vi "file name transfer.vi"(11 "パス":path) -> (0 "file info output":T2, 1 "D con":string, 2 "Experimetal ID":string, 3 "Data file name":string, 4 "F ex Info":T1)   [LabVIEW 2018]
panel:
  out "部分文字列の後 3":string
  out "部分文字列の前":string
  out "部分文字列の後 2":string
  out "EP2 Voltage (mV)":string
  out "EP1 Voltage (mV)":string
  out "Chip ID":string
  out "Ex ID":string
  out "BiasVoltage (mV)":string
  out "Distance (nm)":string
  out "Data form":string
  out "EP2 (mV)":string
  out "EP1 (mV)":string
  out "Target Current (pA)":string
  out "Bias (mV)":string
  out "Distance":string
  out "SW form":string
  out "DAQ time":string
  out "SW Ex name":string
  out "Ex#":string
  out "Sample Name":string
  out "Operator":string
  out "Machine":string
  out "部分文字列の後":string
  out "Ex time":string
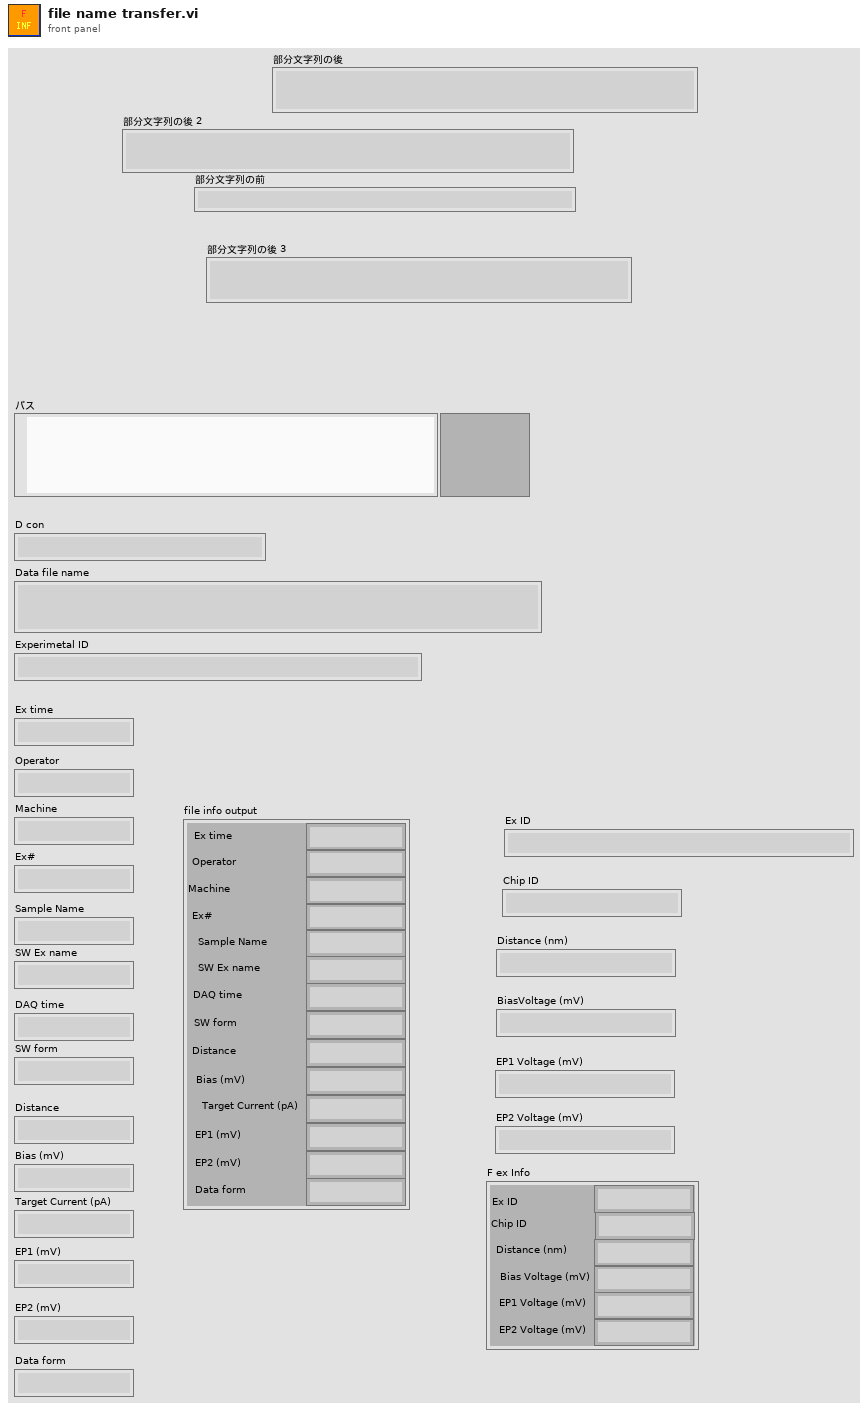
[diagram p1: front panel]
types:
  T1 = cluster{"Ex ID":string, "Chip ID":string, "Distance (nm)":string, "Bias Voltage (mV)":string, "EP1 Voltage (mV)":string, "EP2 Voltage (mV)":string}
  T2 = cluster{"Ex time":string, "Operator":string, "Machine":string, "Ex#":string, "Sample Name":string, "SW Ex name":string, "DAQ time":string, "SW form":string, "Distance":string, "Bias (mV)":string, "Target Current (pA)":string, "EP1 (mV)":string, "EP2 (mV)":string, "Data form":string}
  T3 = cluster{string, string, string, string, string, string, string, string, string, string, string, string, string, string}
  T4 = cluster{string, "Chip ID":string, string, string, string, string}
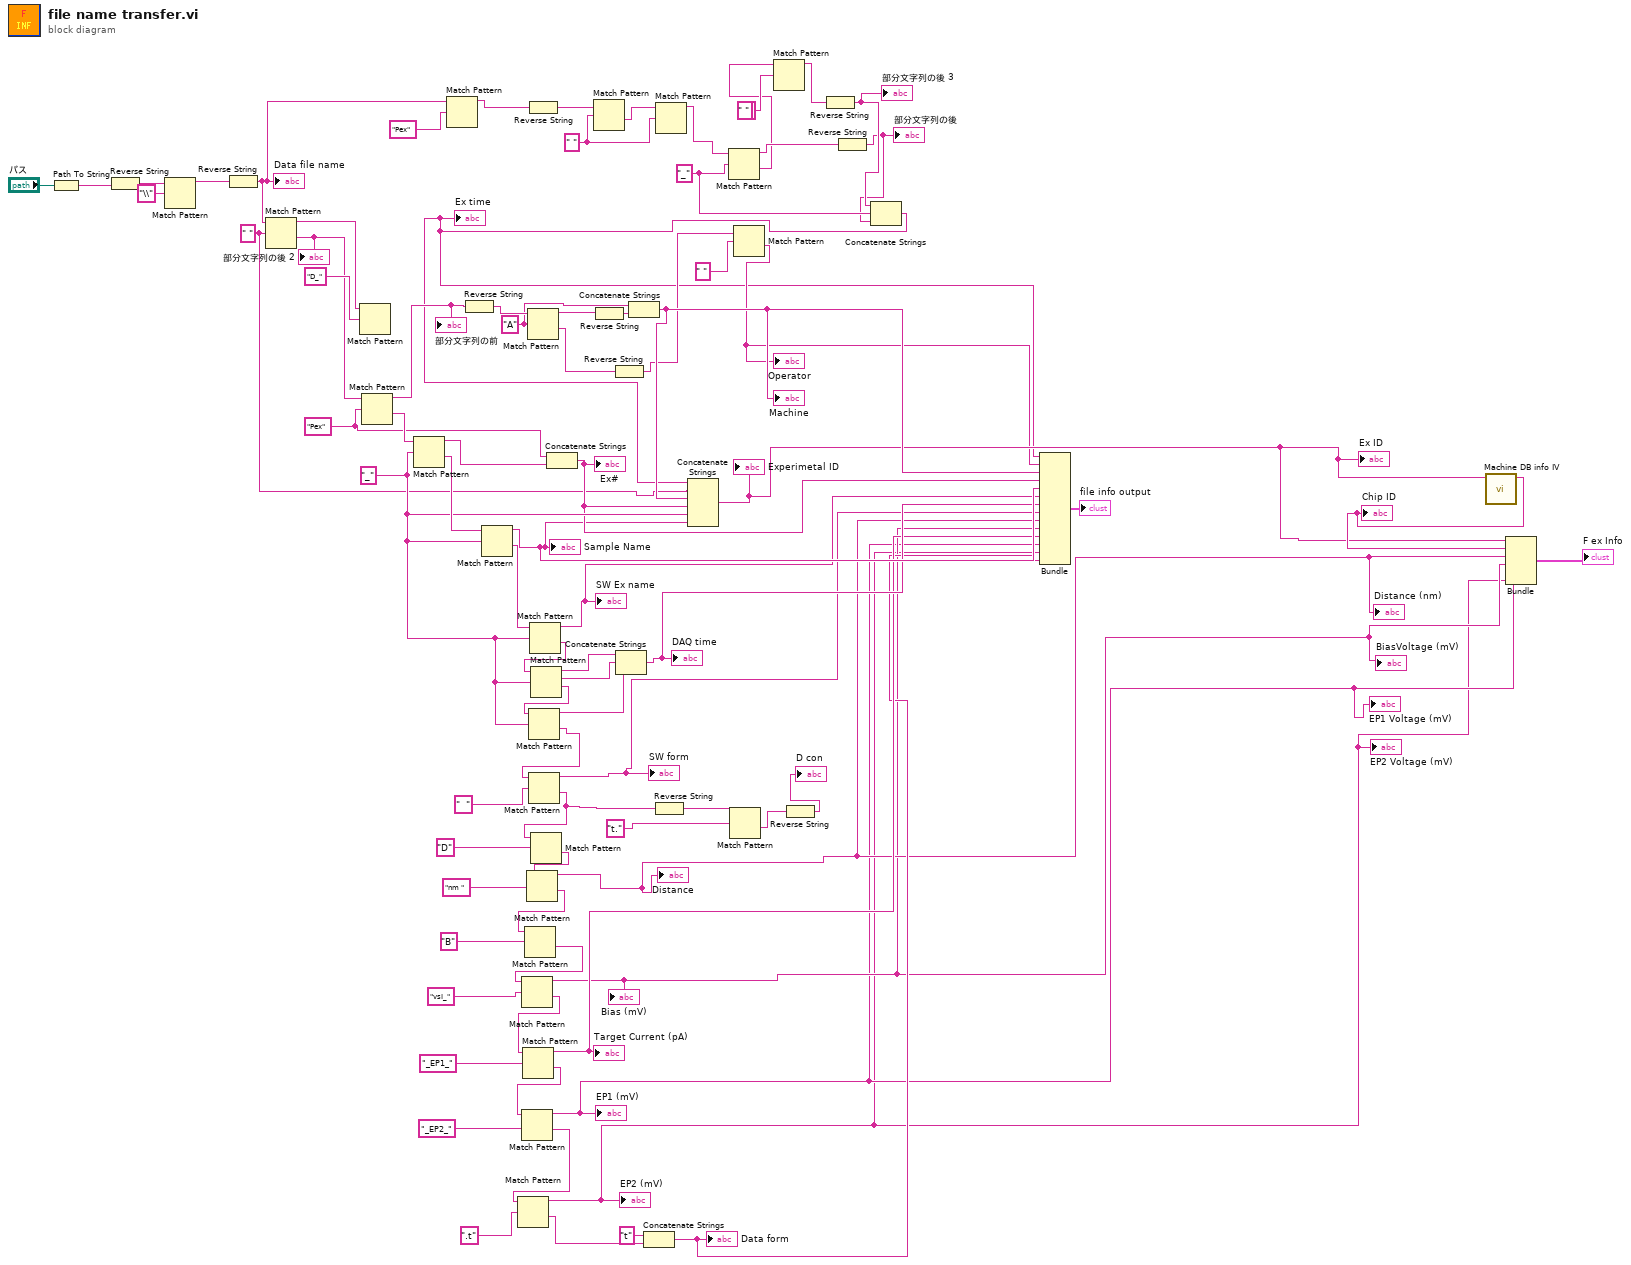
[diagram p0: block diagram]
diagram:
  (unwired) " " ("正規表現")
  w4 = "_" ("string")
  w12 = " " ("正規表現")
  w62 = "_" ("正規表現")
  w71 = "A" ("正規表現")
  w65 = "Pex" ("正規表現")
  w2 = " " ("正規表現")
  n1 = Path To String(path="パス") -> (string=w81:string)
  n2 = Reverse String(1:w81) -> (0:w80:string)
  n3 = Match Pattern(string=w80, regular expression="\\" ("正規表現")) -> (before substring=w78:string)  [unwired: 1 in, 3 out]
  n4 = Reverse String(1:w78) -> (0:w18:string)
  "Data file name" <- w18
  n5 = Match Pattern(string=w18, regular expression=w2) -> (before substring=w77:string, after substring=w75:string)  [unwired: 1 in, 2 out]
  "部分文字列の後 2" <- w75
  n6 = Match Pattern(string=w77, regular expression="D_" ("正規表現")) -> ()  [unwired: 1 in, 4 out]
  n7 = Match Pattern(string=w75, regular expression=w65) -> (before substring=w69:string, after substring=w68:string)  [unwired: 1 in, 2 out]
  "部分文字列の前" <- w69
  n8 = Match Pattern(string=w68, regular expression=w62) -> (before substring=w66:string, after substring=w67:string)  [unwired: 1 in, 2 out]
  n9 = Match Pattern(string=w18, regular expression="Pex" ("正規表現")) -> (before substring=w17:string)  [unwired: 1 in, 3 out]
  n10 = Reverse String(1:w69) -> (0:w74:string)
  n11 = Match Pattern(string=w67, regular expression=w62) -> (before substring=w33:string, after substring=w64:string)  [unwired: 1 in, 2 out]
  "Sample Name" <- w33
  n12 = Reverse String(1:w17) -> (0:w16:string)
  n13 = Match Pattern(string=w74, regular expression=w71) -> (before substring=w73:string, after substring=w70:string)  [unwired: 1 in, 2 out]
  n14 = Match Pattern(string=w64, regular expression=w62) -> (before substring=w32:string, after substring=w61:string)  [unwired: 1 in, 2 out]
  "SW Ex name" <- w32
  n15 = Match Pattern(string=w61, regular expression=w62) -> (before substring=w60:string, match substring=w59:string, after substring=w63:string)  [unwired: 1 in, 1 out]
  n16 = Match Pattern(string=w63, regular expression=w62) -> (before substring=w58:string, after substring=w57:string)  [unwired: 1 in, 2 out]
  n17 = Match Pattern(string=w57, regular expression="  " ("正規表現")) -> (before substring=w30:string, after substring=w46:string)  [unwired: 1 in, 2 out]
  "SW form" <- w30
  n18 = Match Pattern(string=w46, regular expression="D" ("string")) -> (after substring=w53:string)  [unwired: 1 in, 3 out]
  n19 = Match Pattern(string=w53, regular expression="nm " ("文字列")) -> (before substring=w23:string, after substring=w52:string)  [unwired: 1 in, 2 out]
  "Distance" <- w23
  "Distance (nm)" <- w23
  n20 = Match Pattern(string=w52, regular expression="B" ("string")) -> (after substring=w50:string)  [unwired: 1 in, 3 out]
  n21 = Match Pattern(string=w50, regular expression="vsI_" ("string")) -> (before substring=w22:string, after substring=w43:string)  [unwired: 1 in, 2 out]
  "Bias (mV)" <- w22
  "BiasVoltage (mV)" <- w22
  n22 = Match Pattern(string=w43, regular expression="_EP1_" ("文字列")) -> (before substring=w29:string, after substring=w42:string)  [unwired: 1 in, 2 out]
  "Target Current (pA)" <- w29
  n23 = Match Pattern(string=w42, regular expression="_EP2_" ("文字列")) -> (before substring=w21:string, after substring=w39:string)  [unwired: 1 in, 2 out]
  "EP1 (mV)" <- w21
  "EP1 Voltage (mV)" <- w21
  n24 = Match Pattern(string=w39, regular expression=".t" ("文字列")) -> (before substring=w20:string, after substring=w37:string)  [unwired: 1 in, 2 out]
  "EP2 (mV)" <- w20
  "EP2 Voltage (mV)" <- w20
  n25 = Concatenate Strings(w65, w66) -> (w34:string)
  "Ex#" <- w34
  n26 = Match Pattern(string=w16, regular expression=w12) -> (after substring=w11:string)  [unwired: 1 in, 3 out]
  n27 = Reverse String(1:w73) -> (0:w72:string)
  n28 = Reverse String(1:w70) -> (0:w14:string)
  n29 = Concatenate Strings(w60, w59, w58) -> (w31:string)
  "DAQ time" <- w31
  n30 = Concatenate Strings(w71, w72) -> (w35:string)
  "Machine" <- w35
  n31 = Concatenate Strings("t" ("文字列"), w37) -> (w28:string)
  "Data form" <- w28
  n32 = Reverse String(1:w46) -> (0:w45:string)
  n33 = Match Pattern(string=w11, regular expression=w12) -> (before substring=w10:string)  [unwired: 1 in, 3 out]
  n34 = Match Pattern(string=w10, regular expression=w4) -> (before substring=w9:string, after substring=w7:string)  [unwired: 1 in, 2 out]
  n35 = Match Pattern(string=w45, regular expression="t." ("正規表現")) -> (after substring=w48:string)  [unwired: 1 in, 3 out]
  n36 = Match Pattern(string=w14, regular expression=" " ("正規表現")) -> (after substring=w13:string)  [unwired: 1 in, 3 out]
  "Operator" <- w13
  n37 = Match Pattern(string=w7, regular expression="_" ("正規表現")) -> (before substring=w6:string)  [unwired: 1 in, 3 out]
  n38 = Reverse String(1:w48) -> (0:→"D con":string)
  n39 = Reverse String(1:w6) -> (0:w5:string)
  "部分文字列の後 3" <- w5
  n40 = Reverse String(1:w9) -> (0:w3:string)
  "部分文字列の後" <- w3
  n41 = Concatenate Strings(w5, w4, w3) -> (w1:string)
  "Ex time" <- w1
  n42 = Concatenate Strings(w1, w2, w35, w34, w62, w33) -> (w24:string)
  "Experimetal ID" <- w24
  "Ex ID" <- w24
  n43 = Bundle(w1, w13, w35, w34, w33, w32, w31, w30, w23, w22, w29, w21, w20, w28) -> (→"file info output":T3)  [unwired: 1 in]
  n44 = call "Machine DB info IV.vi"("Ex ID"=w24) -> ("Chip ID"=w25:string)  [unwired: 8 in, 2 out]
  "Chip ID" <- w25
  n45 = Bundle(w24, "Chip ID"=w25, w23, w22, w21, w20) -> (→"F ex Info":T4)  [unwired: 1 in]
